vi "IRPID.vi"(3 "error in (no error)":errorcluster, 4 "目標":dbl[](array[numeric])=[0.0, 0.0] format="%#_13g", 5 "Reset":bool) -> (0 "error out":errorcluster, 1 "output":dbl[](array[numeric])=[-0.7554949914993472, -0.03929766619924635], 2 "誤差":dbl[](array[numeric])=[-0.7554949914993472, -0.03929766619924635])   [LabVIEW 2019]
uses:
  <vilib>/addons/control/pid/pid.llb/PID (DBL Array).vi
  <vilib>/addons/control/pid/NI_PID_pid.lvlib
panel:
  in  "dt (s)":dbl=0.01 format="%#_13g"
  out "Waveform Graph":dbl[](graph)=[-0.7554949914993472, -0.03929766619924635]
  out "ENC":dbl[](array[numeric])=[73.0, -142.0]
  in  "PID gains":T1(array[cluster])=[{"proportional gain (Kc)"=5.0, "integral time (Ti, min)"=0.0, "derivative time (Td, min)"=0.0002}, {"proportional gain (Kc)"=5.0, "integral time (Ti, min)"=0.0, "derivative time (Td, min)"=0.0002}] {"derivative time (Td, min)" format="%.4f"; "integral time (Ti, min)" format="%.3f"; "proportional gain (Kc)" format="%.3f"}
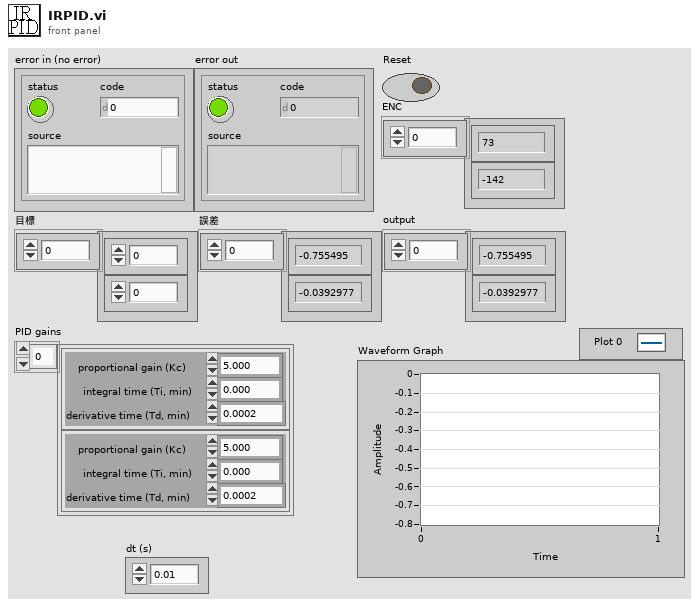
[diagram p1: front panel]
types:
  T1 = cluster{"proportional gain (Kc)":dbl, "integral time (Ti, min)":dbl, "derivative time (Td, min)":dbl}[]
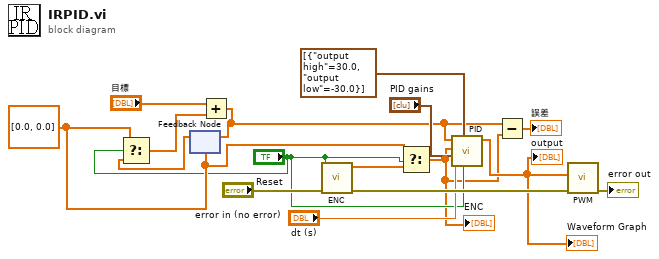
[diagram p0: block diagram]
diagram:
  w4 = dbl[] [0.0, 0.0] ("t")
  n1 = feedback #1(w4) -> (w6:dbl[])
  n2 = Select(t=w4, s="Reset", f=w6) -> (s? t:f=w7:dbl[])
  n3 = Add(x="目標", y=w7) -> (x+y=w5:dbl[])
  n4 = feedback-in #1(w5) -> ()
  n5 = call "ENC.vi"("error in (no error)"="error in (no error)", "Reset"="Reset") -> ("error out"=w15:errorcluster, "ENC"=w3:dbl[])  [unwired: 6 in, 2 out]
  n6 = Select(t=w4, s="Reset", f=w3) -> (s? t:f=w1:dbl[])
  "ENC" <- w1
  n7 = call-poly <vilib>:"PID.vi"("reinitialize? (F)"="Reset", "output range"=cluster{"output high":dbl, "output low":dbl}[] [{"output high"=30.0, "output low"=-30.0}], "dt (s)"="dt (s)", "PID gains"="PID gains", "process variable"=w1, "setpoint"=w5) -> ("output"=w9:dbl[])  [unwired: 4 in, 1 out]
  "output" <- w9
  "Waveform Graph" <- w9
  n8 = Subtract(x=w5, y=w1) -> (x-y=→"誤差":dbl[])
  n9 = call "PWM.vi"("error in (no error)"=w15, "power"=w9) -> ("error out"=→"error out":errorcluster)  [unwired: 9 in]
